vi "Launcher.vi"   [LabVIEW 2024]
panel:
  # "Have 2 pages with the same dependency\ninitialise with dependency\npage 1 can update string\npage 2 initialises with string and can also update string"
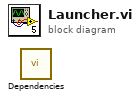
[diagram p0: block diagram]
diagram:
  n1 = call "Dependencies.vi"() -> ()  [unwired: 11 in, 1 out]
